vi "update_providers.vi"(8 "error in (no error)":errorcluster, 10 "log_entry":T1 {"datetime" format="%<%x %.3X>T"}, 11 "system.logging in":refnum<class "system.logging.lvclass">) -> (0 "error out":errorcluster, 3 "system.logging out":refnum<class "system.logging.lvclass">)   [LabVIEW 2021, in "system.logging.lvclass"]
uses:
  system.logging.lvclass
  log_entry.ctl
  severity.ctl
  system.logging.lvclass/system.logging.ctl
  system.logging.provider/system.logging.provider.lvclass/system.logging.provider.ctl
  system.logging.provider/system.logging.provider.lvclass
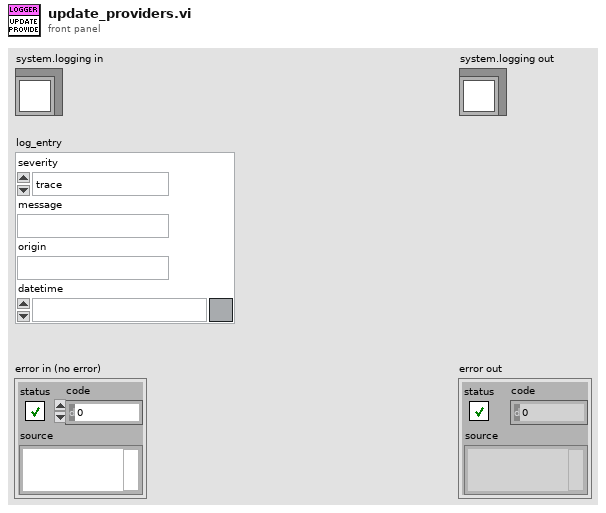
[diagram p1: front panel]
types:
  T1 = typedef "system.logging.lvclass/log_entry.ctl" = cluster{"severity":T2, "message":string, "origin":string, "datetime":timestamp}
  T2 = typedef "system.logging.lvclass/severity.ctl" = enum8{"trace", "debug", "info", "warning", "error"}
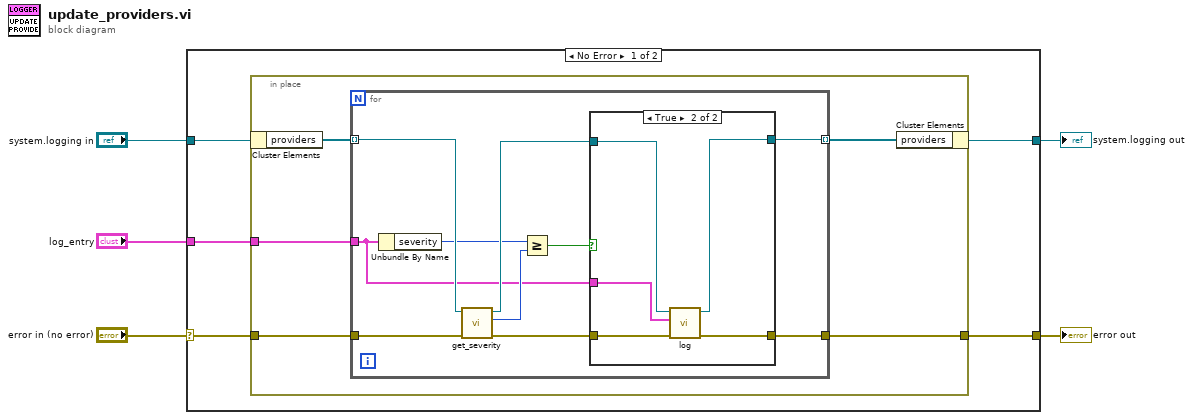
[diagram p0: block diagram]
diagram:
  n1 = case shown="No Error" "error in (no error)" {
    selector: "error in (no error)" -> [w8 w34]
    tunnel: [w7 w34] -> w4
    tunnel: [w6 w33] -> w2
    tunnel: "system.logging in" -> [w10 w33]
    tunnel: "log_entry" -> [w9 _]
    frame No Error {
      n2 = in-place {
        in-place-border: w9 -> [w14]
        in-place-border: w8 -> [w13]
        in-place-border: [w11] -> w7
        n3 = in-place-cluster #1(w10) -> ("providers"=w15:refnum<class "system.logging.provider.lvclass">[])
        n4 = for {
          tunnel: w15 -> [w22] mode=indexing
          tunnel: w14 -> [w16]
          tunnel: w13 -> [w23]
          tunnel: [w25] -> w12 mode=indexing
          tunnel: [w24] -> w11
          n5 = Unbundle By Name(w16) -> ("severity"=w20:T2)
          n6 = call "get_severity.vi"("error in (no error)"=w23, "system.logging.provider in"=w22) -> ("error out"=w17:errorcluster, "severity"=w19:T2, "system.logging.provider out"=w21:refnum<class "system.logging.provider.lvclass">)  [unwired: 7 in]
          n7 = Greater Or Equal?(x=w20, y=w19) -> (x >= y?=w18:bool)
          n8 = case shown="True" w18 {
            tunnel: [w27 w32] -> w25
            tunnel: [w26 w31] -> w24
            tunnel: w21 -> [w27 w30]
            tunnel: w17 -> [w26 w29]
            tunnel: w16 -> [_ w28]
            frame False {
            }
            frame True {
              n9 = call-dynamic "log.vi"("error in (no error)"=w29, "log_entry"=w28, "system.logging.provider in"=w30) -> ("error out"=w31:errorcluster, "system.logging.provider out"=w32:refnum<class "system.logging.provider.lvclass">)  [unwired: 7 in]
            }
          }
        }
        n10 = in-place-cluster #1("providers"=w12) -> (w6:refnum<class "system.logging.lvclass">)
      }
    }
    frame Error {
    }
  }
  "error out" <- w4
  "system.logging out" <- w2
